vi "GetElements(Multiple).vi"(7 "Qualified Name":string, 8 "error in (no error)":errorcluster, 10 "keys":string[](array[string]), 11 "ConfigManager in":refnum<class "ConfigManager.lvclass">) -> (0 "error out":errorcluster, 1 "Values":string[](array[string]), 2 "Keys":string[](array[string]), 3 "ConfigManager out":refnum<class "ConfigManager.lvclass">, 4 "Found":bool[](array[boolean]))   [LabVIEW 2013, in "CfgManager.lvlib" / "ConfigManager.lvclass"]
uses:
  ConfigManager.lvclass
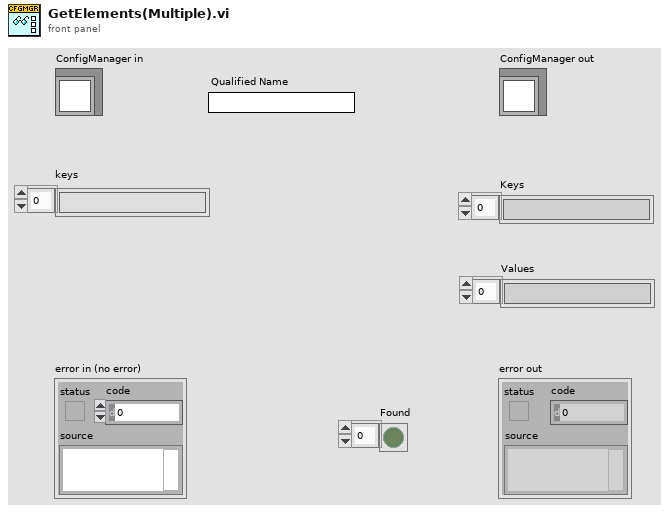
[diagram p1: front panel]
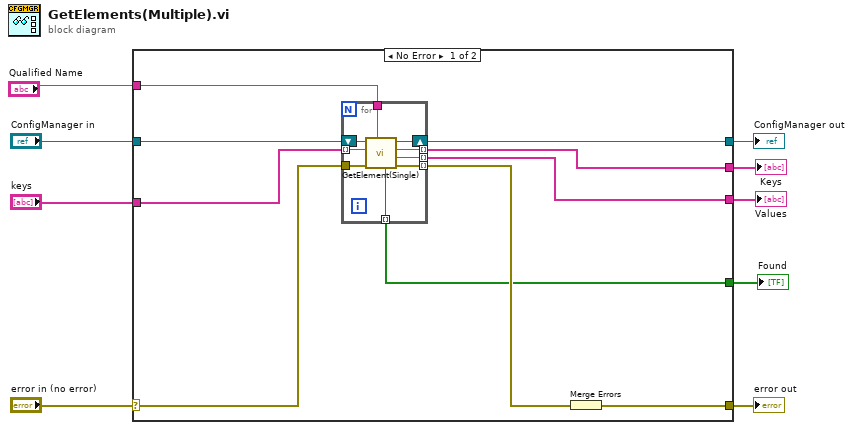
[diagram p0: block diagram]
diagram:
  n1 = case shown="No Error" "error in (no error)" {
    selector: "error in (no error)" -> [w16 w30]
    tunnel: [w14 w30] -> w8
    tunnel: [w18 w29] -> w6
    tunnel: "ConfigManager in" -> [w19 w29]
    tunnel: "keys" -> [w17 _]
    tunnel: [w11 _] -> w4
    tunnel: [w12 _] -> w3
    tunnel: "Qualified Name" -> [w13 _]
    tunnel: [w10 _] -> w1
    frame No Error {
      n2 = for {
        tunnel: w17 -> [w26] mode=indexing
        tunnel: [w25] -> w10 mode=indexing
        tunnel: w16 -> [w24]
        tunnel: [w23] -> w15 mode=indexing
        shift-right: [w27] -> w18
        shift-left: w19 -> [w28]
        tunnel: [w22] -> w11 mode=indexing
        tunnel: w13 -> [w21]
        tunnel: [w20] -> w12 mode=indexing
        n3 = call-dynamic "GetElement(Single).vi"("Qualified Name"=w21, "error in (no error)"=w24, "Key"=w26, "ConfigManager in"=w28) -> ("error out"=w23:errorcluster, "Value"=w22:string, "Key"=w25:string, "ConfigManager out"=w27:refnum<class "ConfigManager.lvclass">, "found"=w20:bool)  [unwired: 3 in]
      }
      n4 = Merge Errors(w15) -> (w14:errorcluster)
    }
    frame Error {
    }
  }
  "error out" <- w8
  "ConfigManager out" <- w6
  "Values" <- w4
  "Found" <- w3
  "Keys" <- w1
